vi "Convert Error Core.vi"(8 "error in (no error)":errorcluster, 11 "return type":i32) -> (0 "error out":errorcluster)   [LabVIEW 2021, in "Iceoryx.lvlib"]
uses:
  Iceoryx.lvlib
  <vilib>/CIF Foundation/CIF Utilities/Errors/Errors_CIF_U.lvlib
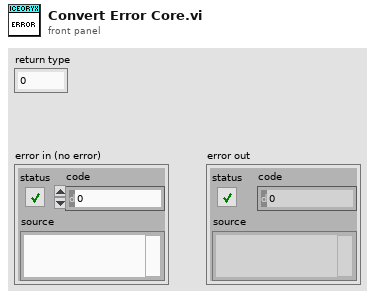
[diagram p1: front panel]
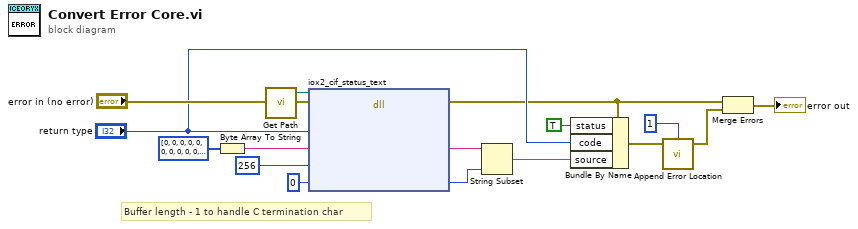
[diagram p0: block diagram]
diagram:
  # "Buffer length - 1 to handle C termination char"
  n1 = Byte Array To String(unsigned byte array=u8[] [0, 0, 0, 0, 0, 0, 0, 0, 0, 0, 0, 0, 0, 0, 0, 0, 0, 0, 0, 0, 0, 0, 0, 0, 0, 0, 0, 0, 0, 0, 0, 0, 0, 0, 0, 0, 0, 0, 0, 0, 0, 0, 0, 0, 0, 0, 0, 0, 0, 0, 0, 0, 0, 0, 0, 0, 0, 0, 0, 0, 0, 0, 0, 0, 0, 0, 0, 0, 0, 0, 0, 0, 0, 0, 0, 0, 0, 0, 0, 0, 0, 0, 0, 0, 0, 0, 0, 0, 0, 0, 0, 0, 0, 0, 0, 0, 0, 0, 0, 0, 0, 0, 0, 0, 0, 0, 0, 0, 0, 0, 0, 0, 0, 0, 0, 0, 0, 0, 0, 0, 0, 0, 0, 0, 0, 0, 0, 0, 0, 0, 0, 0, 0, 0, 0, 0, 0, 0, 0, 0, 0, 0, 0, 0, 0, 0, 0, 0, 0, 0, 0, 0, 0, 0, 0, 0, 0, 0, 0, 0, 0, 0, 0, 0, 0, 0, 0, 0, 0, 0, 0, 0, 0, 0, 0, 0, 0, 0, 0, 0, 0, 0, 0, 0, 0, 0, 0, 0, 0, 0, 0, 0, 0, 0, 0, 0, 0, 0, 0, 0, 0, 0, 0, 0, 0, 0, 0, 0, 0, 0, 0, 0, 0, 0, 0, 0, 0, 0, 0, 0, 0, 0, 0, 0, 0, 0, 0, 0, 0, 0, 0, 0, 0, 0, 0, 0, 0, 0, 0, 0, 0, 0, 0, 0, 0, 0, 0, 0, 0, 0, 0, 0, 0, 0, 0, 0, 0]) -> (string=w12:string)
  n2 = call "Get Path.vi"() -> ("libiox2_cif path"=w11:path)  [unwired: 4 in]
  n3 = dll-call lib="D:/dev/iceoryx2_lvwrapper/dist/iox2_cif.dll" fn="iox2_cif_status_text"(path in=w11, error in="error in (no error)", "status"="return type", "buf"=w12, "buf_len"=u32 256 ("max_count"), "out_len"=u32 0 ("actual")) -> (error out=w3:errorcluster, "buf"=w10:string, "out_len"=w9:u32)  [unwired: 4 in, 1 out]
  n4 = String Subset(string=w10, length (rest)=w9) -> (substring=w7:string)  [unwired: 1 in]
  n5 = Bundle By Name(cluster=w3, "status"=TRUE, "code"="return type", "source"=w7) -> (w4:errorcluster)
  n6 = call <vilib>:"Append Error Location.vi"("error in (no error)"=w4, "Chain Depth"=1) -> ("error out"=w2:errorcluster)  [unwired: 3 in]
  n7 = Merge Errors(w3, w2) -> (→"error out":errorcluster)
